vi "RT Main.vi"() -> ()   [LabVIEW 2016]
doc: "This template is for the Queued Message Handler design pattern.\n\nThe Event Handling Loop generates messages based on user interface actions.\n\nThe Message Handling Loop processes messages generated by the Event Handling Loop, or by other messages. The messages are string values, so new messages can be added easily to the Message Cases case structure in the Message Handling Loop. Each message cluster can also provide an optional value for Message Data, which is a variant that can be converted to whatever message-specific data is required."
uses:
  Globals/Global - All RT Loop Stop.vi
  Globals/Global - Monitoring Variables.vi
  Globals/Global - Configuration Options.vi
  Globals/Global - RT Stream Connections.vi
  <vilib>/FPGAPlugInAG/cRIO-9068/niLvFpga_Open_cRIO-9068.vi
  <vilib>/rvi/interface/common/dynamic/niFpgaDynamicAddResources.vi
  <vilib>/FPGAPlugInAG/Dynamic/niLvFpga_Reset_Dynamic.vi
  <vilib>/rvi/errors/niLvFpgaAdjustHostInterfaceError.vi
  <vilib>/FPGAPlugInAG/Dynamic/niLvFpga_Run_Dynamic.vi
  <vilib>/rvi/interface/nirviOpenFPGA/nirviOpenFPGA.xnode
  FPGA Bitfiles/v1.1.10032017CSU_FPGATarget2_FPGAMain_uXAbGLR-yyg.lvbitx
  FPGA Main.vi
  <vilib>/rvi/interface/nirviMethod/nirviMethod.xnode
  <vilib>/rvi/interface/nirviReadWriteControl/nirviReadWriteControl.xnode
  support/Message Queue/Message Queue.lvlib
  <vilib>/nisyscfg/nisyscfg.lvlib
  <vilib>/rvi/interface/Simulation/niFpgaSimulationCallBeginRW.vi
  NiFpgaLv.dll
panel:
  in  "error in (no error)":errorcluster
  # "Programa que contém a rotina principal do sistema.\nRoda todos os 4 loops principais;\nAquisição e armazenamento;\nSaúde do sistema e monitoramento da FPGA;\nComandos da interface de usuário;\nWatchdog.\n\nTambém contém a chamada para etapa de Transmissão, referente ao módulo NI 9269."
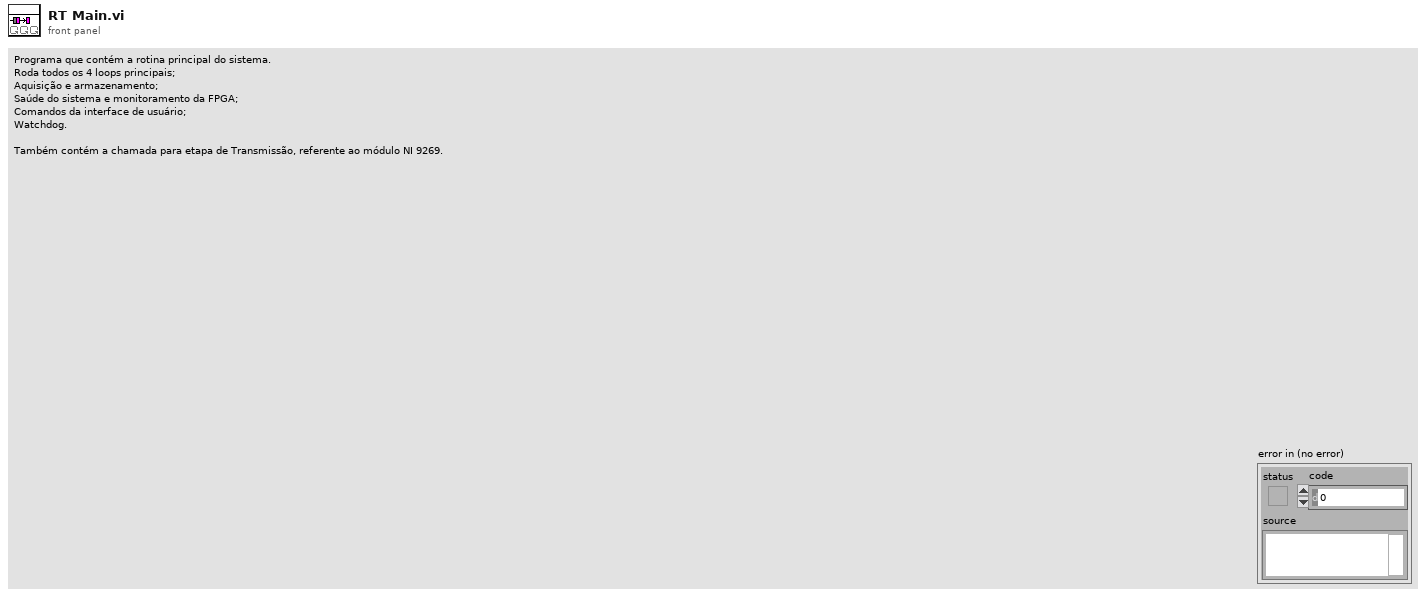
[diagram p1: front panel]
types:
  T1 = typedef "Acquisition and Logging Configuration.ctl" = cluster{"Data Rate":T2, "Samples per Read":i32, "Number of Reads to Save":i32, "Data File Name":string, "TDMS Properties":T3[], "Number of Channels":i32, "Channel Scale Array":fxp<+,24,12>[], "Channel Names":string[], "Trigger - RMS Value":dbl, "Trigger - Channel":i32, "Trigger - Time (Minute)":i32, "Frequency ":i32, "Amplitude (0~10)":dbl}
  T2 = typedef "nicrio_cRIO-9239_DataRatesRing.ctl" = u8
  T3 = typedef "TDMS Properties.ctl" = cluster{"Name":string, "Value":string}
  T4 = typedef "Message Queue.lvlib/All Real-Time Message Queues.ctl" = cluster{"Message Handler":refnum<queue>, "Acquisition and Logging":refnum<queue>}
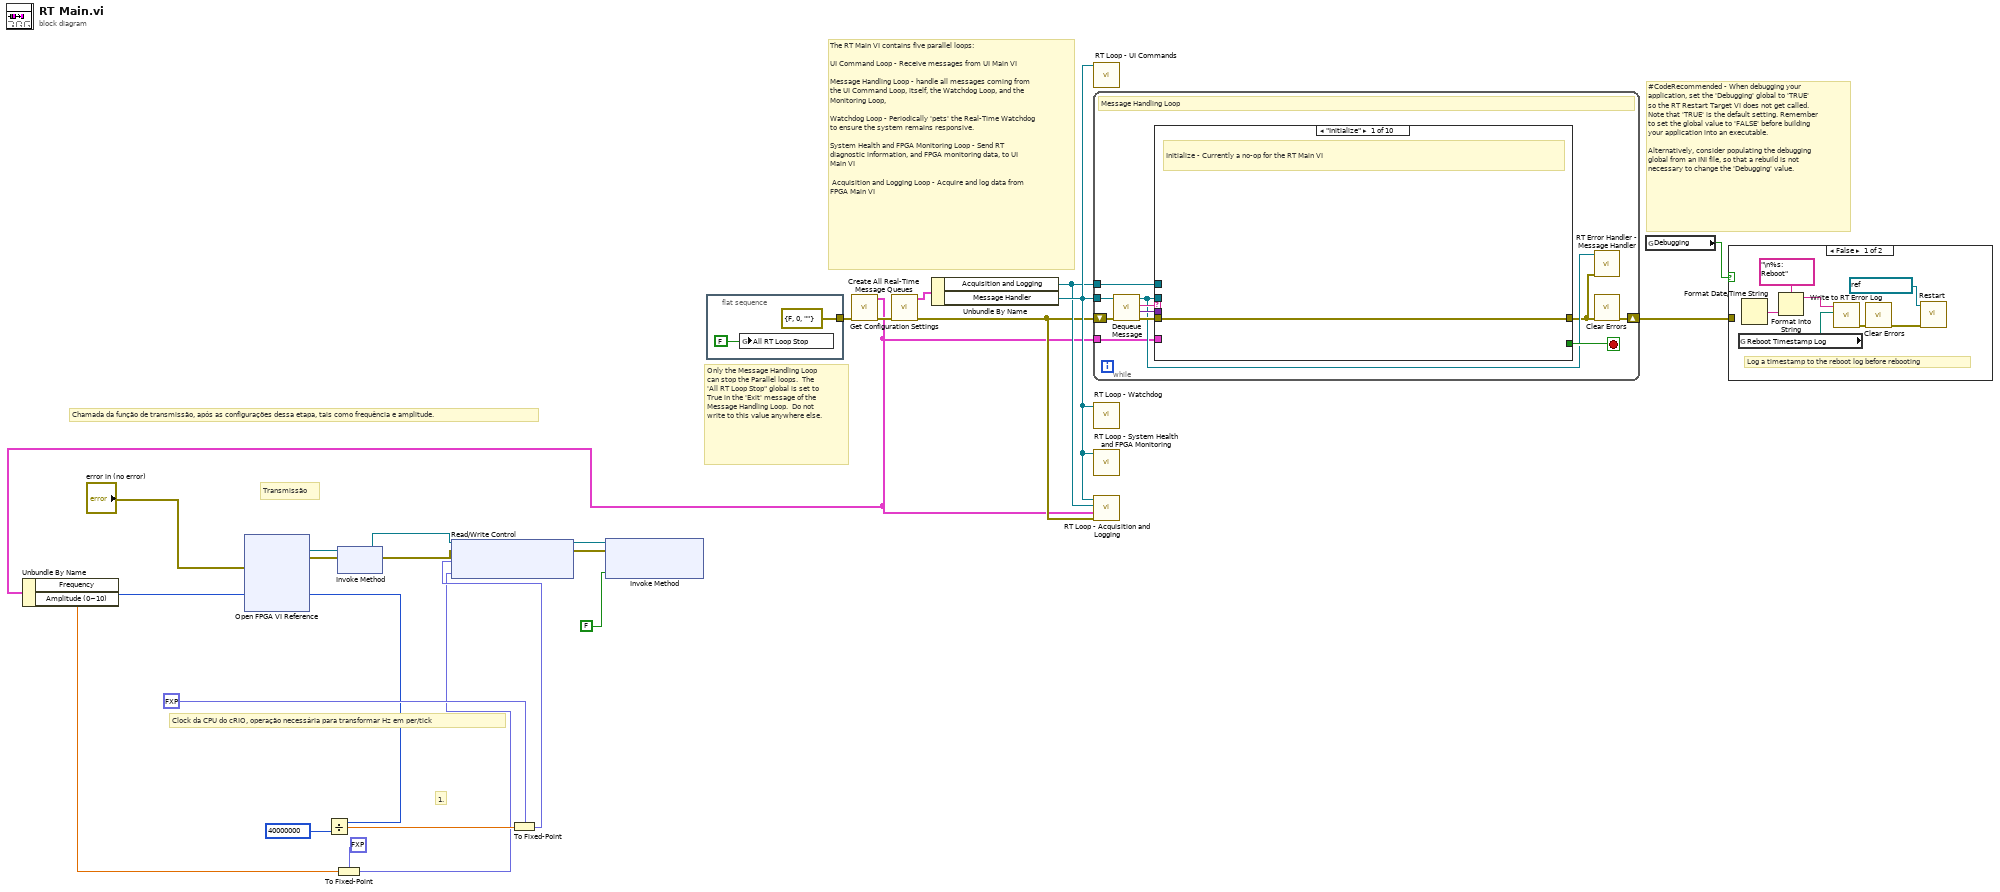
[diagram p0: block diagram]
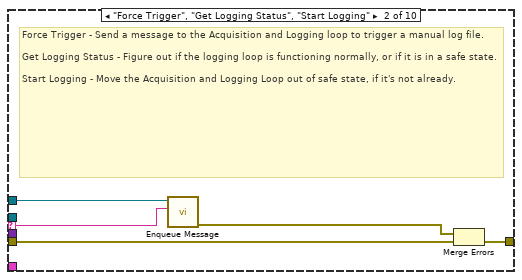
[diagram p3: hidden frame]
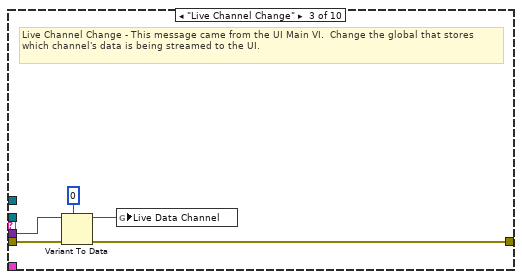
[diagram p4: hidden frame]
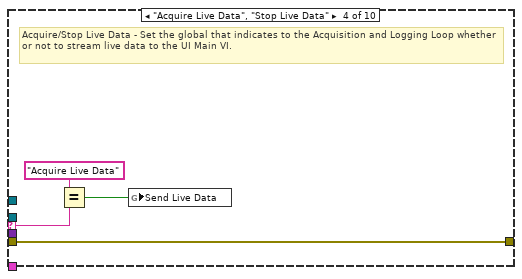
[diagram p5: hidden frame]
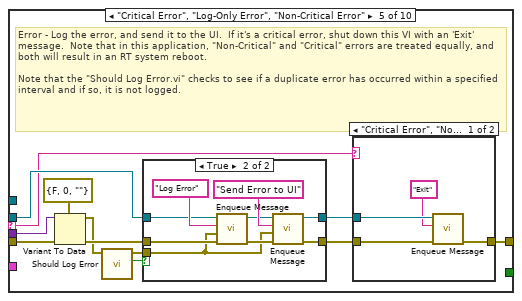
[diagram p6: hidden frame]
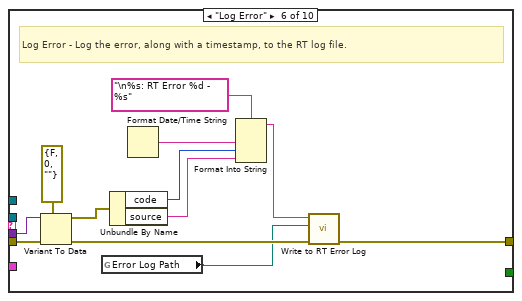
[diagram p9: hidden frame]
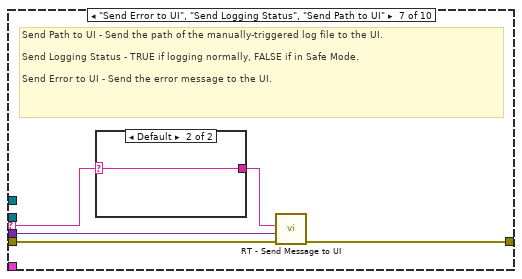
[diagram p10: hidden frame]
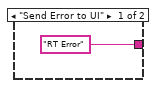
[diagram p11: hidden frame]
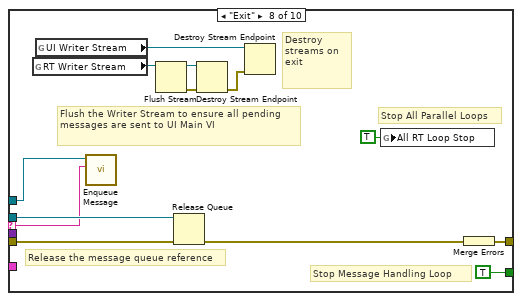
[diagram p12: hidden frame]
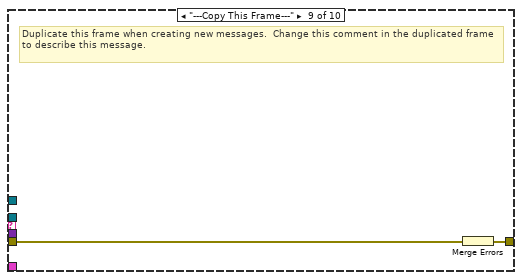
[diagram p13: hidden frame]
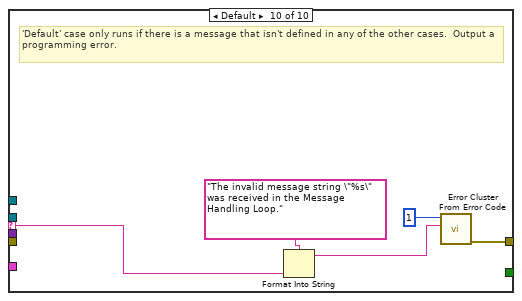
[diagram p14: hidden frame]
diagram:
  # "Chamada da função de transmissão, após as configurações dessa etapa, tais como frequência e amplitude."
  # "Transmissão"
  # "Clock da CPU do cRIO, operação necessária para transformar Hz em per/tick"
  # "1."
  # "#CodeRecommended - When debugging your application, set the 'Debugging' global to 'TRUE' so the RT Restart Target VI does not get called.  Note that 'TRUE' is the default setting. Remember to set the global value to 'FALSE' before building your application into an executable.\n\nAlternatively, consider populating the debugging global from an INI file, so that a rebuild is not necessary to change the 'Debugging' value."
  # "The RT Main VI contains five parallel loops:\n\nUI Command Loop - Receive messages from UI Main VI\n\nMessage Handling Loop - handle all messages coming from the UI Command Loop, itself, the Watchdog Loop, and the Monitoring Loop, \n\nWatchdog Loop - Periodically 'pets' the Real-Time Watchdog to ensure the system remains responsive.\n\nSystem Health and FPGA Monitoring Loop - Send RT diagnostic information, and FPGA monitoring data, to UI Main VI\n\n Acquisition and Logging Loop - Acquire and log data from FPGA Main VI"
  # "Only the Message Handling Loop can stop the Parallel loops.  The 'All RT Loop Stop\" global is set to True in the 'Exit' message of the Message Handling Loop.  Do not write to this value anywhere else."
  n1 = xnode "Open FPGA VI Reference"("error in"="error in (no error)") -> ("FPGA VI Reference Out"=w3:refnum<k20>, "error out"=w2:errorcluster)  [unwired: 1 in]
  n2 = xnode "Invoke Method"("FPGA VI Reference In"=w3, "error in"=w2) -> ("FPGA VI Reference Out"=w4:refnum<k20>, "error out"=w1:errorcluster)
  n3 = flat-sequence {
    tunnel: [errorcluster {"status"=FALSE, "code"=0, "source"=""} ("error constant")] -> w25
    frame #0 {
      n4 = global write "Global - All RT Loop Stop.vi" "All RT Loop Stop"(FALSE) -> ()
    }
  }
  n5 = call "Get Configuration Settings.vi"("error in (no error)"=w25) -> ("error out"=w22:errorcluster, "Acquisition and Logging Configuration"=w7:T1)  [unwired: 9 in]
  n6 = Unbundle By Name(w7) -> ("Frequency"=w5:i32, "Amplitude (0~10)"=w6:dbl)
  n7 = Divide(x=w5, y=40000000) -> (x/y=w15:dbl)
  n8 = To Fixed-Point(fixed-point type=fxp<+/-,20,5> 0.0, number=w6) -> (fixed-point=w12:fxp<+/-,20,5>)
  n9 = To Fixed-Point(fixed-point type=fxp<+,32,0> 0.0, number=w15) -> (fixed-point=w13:fxp<+,32,0>)
  n10 = xnode "Read/Write Control"("FPGA VI Reference In"=w4, "error in"=w1, "Frequency (periods/tick)"=w13, "Amplitude"=w12) -> ("FPGA VI Reference Out"=w11:refnum<k20>, "error out"=w10:errorcluster)
  n11 = xnode "Invoke Method"("FPGA VI Reference In"=w11, "error in"=w10, "Wait Until Done (F)"=FALSE) -> ()  [unwired: 2 out]
  n12 = call "Create All Real-Time Message Queues.vi"("error in (no error)"=w22) -> ("error out"=w18:errorcluster, "Message Queues out"=w20:T4)  [unwired: 9 in]
  n13 = Unbundle By Name(w20) -> ("Acquisition and Logging"=w19:refnum<queue>, "Message Handler"=w21:refnum<queue>)
  n14 = call "RT Loop - UI Commands.vi"("Message Queue"=w21) -> ()  [unwired: 11 in]
  n15 = while {
    tunnel: w21 -> [w33]
    shift-right: [w31] -> w24
    shift-left: w18 -> [w37]
    tunnel: w19 -> [w29]
    tunnel: w7 -> [w28]
    stop <- w38 stop-if-true
    # "Message Handling Loop"
    n16 = call "Dequeue Message.vi"("error in (no error)"=w37, "Message Queue"=w33) -> ("error out"=w36:errorcluster, "Message Data"=w34:variant, "Message"=w35:string, "dup Message Queue"=w32:refnum<queue>)  [unwired: 6 in]
    n17 = case "Message Cases" shown="\"Initialize\"" w35 {
      selector: w35 -> [_ w42 _ w52 w59 _ w95 w103 _ w119]
      tunnel: w32 -> [_ _ _ _ w60 _ _ w113 _ _]
      tunnel: w36 -> [w39 w44 w49 w53 w62 w93 w98 w109 w115 _]
      tunnel: [w39 w41 w48 w53 w65 w84 w97 w110 w114 w117] -> w30
      tunnel: [_ _ _ _ _ _ _ TRUE _ _] -> w38
      tunnel: w34 -> [_ _ w47 _ w54 w92 w96 _ _ _]
      tunnel: w29 -> [_ w43 _ _ _ _ _ w104 _ _]
      tunnel: w28 -> [_ _ _ _ _ _ _ _ _ _]
      frame "Initialize" {
        # "Initialize - Currently a no-op for the RT Main VI"
      }
      frame "Force Trigger", "Get Logging Status", "Start Logging" {
        # "Force Trigger - Send a message to the Acquisition and Logging loop to trigger a manual log file.\n\nGet Logging Status - Figure out if the logging loop is functioning normally, or if it is in a safe state.\n\nStart Logging - Move the Acquisition and Logging Loop out of safe state, if it's not already."
        n18 = call "Enqueue Message.vi"("Message"=w42, "Message Queue"=w43) -> ("error out"=w40:errorcluster)  [unwired: 8 in, 1 out]
        n19 = Merge Errors(w40, w44) -> (w41:errorcluster)
      }
      frame "Live Channel Change" {
        # "Live Channel Change - This message came from the UI Main VI.  Change the global that stores which channel's data is being streamed to the UI."
        n20 = Variant To Data(error in=w49, type=u32 0, Variant=w47) -> (data=w45:u32, error out=w48:errorcluster)
        n21 = global write "Global - Monitoring Variables.vi" "Live Data Channel"(w45) -> ()
      }
      frame "Acquire Live Data", "Stop Live Data" {
        # "Acquire/Stop Live Data - Set the global that indicates to the Acquisition and Logging Loop whether or not to stream live data to the UI Main VI."
        n22 = Equal?(x="Acquire Live Data", y=w52) -> (x = y?=w50:bool)
        n23 = global write "Global - Monitoring Variables.vi" "Send Live Data"(w50) -> ()
      }
      frame "Critical Error", "Log-Only Error", "Non-Critical Error" {
        # "Error - Log the error, and send it to the UI.  If it's a critical error, shut down this VI with an 'Exit' message.  Note that in this application, \"Non-Critical\" and \"Critical\" errors are treated equally, and both will result in an RT system reboot.\n\nNote that the \"Should Log Error.vi\" checks to see if a duplicate error has occurred within a specified interval and if so, it is not logged."
        n24 = Variant To Data(error in=w62, type=errorcluster {"status"=FALSE, "code"=0, "source"=""} ("error out"), Variant=w54) -> (data=w57:errorcluster, error out=w63:errorcluster)
        n25 = call "Should Log Error.vi"("error to report"=w57) -> ("Should Log Error?"=w55:bool, "dup error to report"=w56:errorcluster)  [unwired: 9 in]
        n26 = case shown="True" w55 {
          tunnel: [w67 w74] -> w61
          tunnel: [w66 w73] -> w58
          tunnel: w60 -> [w66 w72]
          tunnel: w63 -> [w67 w69]
          tunnel: w56 -> [_ w68]
          frame False {
          }
          frame True {
            n27 = call "Enqueue Message.vi"("error in (no error)"=w69, "Message Data"=w68, "Message"="Log Error", "Message Queue"=w72) -> ("error out"=w70:errorcluster, "dup Message Queue"=w71:refnum<queue>)  [unwired: 6 in]
            n28 = call "Enqueue Message.vi"("error in (no error)"=w70, "Message Data"=w68, "Message"="Send Error to UI", "Message Queue"=w71) -> ("error out"=w74:errorcluster, "dup Message Queue"=w73:refnum<queue>)  [unwired: 6 in]
          }
        }
        n29 = case shown="\"Critical Error\", \"Non-Critical Error\"" w59 {
          tunnel: w61 -> [w80 w81]
          tunnel: w58 -> [w78 _]
          tunnel: [w79 w81] -> w65
          frame "Critical Error", "Non-Critical Error" {
            n30 = call "Enqueue Message.vi"("error in (no error)"=w80, "Message"="Exit", "Message Queue"=w78) -> ("error out"=w79:errorcluster)  [unwired: 7 in, 1 out]
          }
          frame Default {
          }
        }
      }
      frame "Log Error" {
        # "Log Error - Log the error, along with a timestamp, to the RT log file."
        n31 = Variant To Data(error in=w93, type=errorcluster {"status"=FALSE, "code"=0, "source"=""} ("error constant"), Variant=w92) -> (data=w87:errorcluster, error out=w90:errorcluster)
        n32 = global read "Global - Configuration Options.vi" "Error Log Path"() -> (w82:path)
        n33 = Unbundle By Name(w87) -> ("code"=w86:i32, "source"=w85:string)
        n34 = Format Date/Time String() -> (date/time string=w88:string)  [unwired: 3 in]
        n35 = Format Into String(format string="\n%s: RT Error %d - %s", w88, w86, w85) -> (resulting string=w83:string)  [unwired: 2 in, 1 out]
        n36 = call "Write to RT Error Log.vi"("error in (no error)"=w90, "Error Log Path"=w82, "Log Entry"=w83) -> ("error out"=w84:errorcluster)  [unwired: 8 in]
      }
      frame "Send Error to UI", "Send Logging Status", "Send Path to UI" {
        # "Send Path to UI - Send the path of the manually-triggered log file to the UI.\n\nSend Logging Status - TRUE if logging normally, FALSE if in Safe Mode.\n\nSend Error to UI - Send the error message to the UI."
        n37 = case shown="Default" w95 {
          selector: w95 -> [_ w100]
          tunnel: ["RT Error" ("Message") w100] -> w94
          frame "Send Error to UI" {
          }
          frame Default {
          }
        }
        n38 = call "RT - Send Message to UI.vi"("error in (no error)"=w98, "Message Data"=w96, "Message"=w94) -> ("error out"=w97:errorcluster)  [unwired: 8 in]
      }
      frame "Exit" {
        # "Flush the Writer Stream to ensure all pending messages are sent to UI Main VI"
        # "Destroy streams on exit"
        # "Stop Message Handling Loop"
        # "Stop All Parallel Loops"
        # "Release the message queue reference"
        n39 = global read "Global - RT Stream Connections.vi" "RT Writer Stream"() -> (w107:refnum<k21>)
        n40 = global read "Global - RT Stream Connections.vi" "UI Writer Stream"() -> (w106:refnum<k21>)
        n41 = call "Enqueue Message.vi"("Message"=w103, "Message Queue"=w104) -> ()  [unwired: 8 in, 2 out]
        n42 = Flush Stream(11:w107) -> (0:w101:errorcluster, 3:w102:refnum<k21>)  [unwired: 3 in, 1 out]
        n43 = Release Queue(queue=w113, error in (no error)=w109) -> (error out=w111:errorcluster)  [unwired: 1 in, 2 out]
        n44 = Destroy Stream Endpoint(8:w101, 11:w102) -> (0:w105:errorcluster)
        n45 = Destroy Stream Endpoint(8:w105, 11:w106) -> ()  [unwired: 1 out]
        n46 = global write "Global - All RT Loop Stop.vi" "All RT Loop Stop"(TRUE ("Stop Monitoring Loops")) -> ()
        n47 = Merge Errors(w111) -> (w110:errorcluster)
      }
      frame "---Copy This Frame---" {
        # "Duplicate this frame when creating new messages.  Change this comment in the duplicated frame to describe this message."
        n48 = Merge Errors(w115) -> (w114:errorcluster)
      }
      frame Default {
        # "'Default' case only runs if there is a message that isn't defined in any of the other cases.  Output a programming error."
        n49 = Format Into String(format string="The invalid message string \"%s\" was received in the Message Handling Loop." ("Unknown Message Error Text"), w119) -> (resulting string=w116:string)  [unwired: 2 in, 1 out]
        n50 = call <vilib>:"Error Cluster From Error Code.vi"("error message (\"\")"=w116, "error code (0)"=1) -> ("error out"=w117:errorcluster)  [unwired: 7 in]
      }
    }
    n51 = call "RT Error Handler - Message Handler.vi"("error in (no error)"=w30, "Message Queue"=w32) -> ()  [unwired: 9 in, 1 out]
    n52 = call <vilib>:"Clear Errors.vi"("error in (no error)"=w30) -> ("error out"=w31:errorcluster)  [unwired: 5 in, 1 out]
  }
  n53 = call "RT Loop - Watchdog.vi"("Message Queue"=w21) -> ()  [unwired: 11 in]
  n54 = call "RT Loop - System Health and FPGA Monitoring.vi"("Message Queue"=w21) -> ()  [unwired: 11 in]
  n55 = call "RT Loop - Acquisition and Logging.vi"("error in (no error)"=w18, "Acquisition and Logging Configuration"=w7, "Acquisition and Logging Queue"=w19, "Message Queue"=w21) -> ()  [unwired: 8 in]
  n56 = global read "Global - Configuration Options.vi" "Debugging"() -> (w23:bool)
  n57 = case shown="False" w23 {
    tunnel: w24 -> [_ _]
    frame False {
      # "Log a timestamp to the reboot log before rebooting"
      n58 = global read "Global - Configuration Options.vi" "Reboot Timestamp Log"() -> (w123:path)
      n59 = Format Date/Time String() -> (date/time string=w125:string)  [unwired: 3 in]
      n60 = Format Into String(format string="\n%s: Reboot", w125) -> (resulting string=w124:string)  [unwired: 2 in, 1 out]
      n61 = call "Write to RT Error Log.vi"("Error Log Path"=w123, "Log Entry"=w124) -> ("error out"=w127:errorcluster)  [unwired: 9 in]
      n62 = call <vilib>:"Clear Errors.vi"("error in (no error)"=w127) -> ("error out"=w122:errorcluster)  [unwired: 5 in, 1 out]
      n63 = call <vilib>:"Restart.vi"("error in (no error)"=w122, "Session in"=refnum<k21> "localhost" ("session in")) -> ()  [unwired: 7 in, 3 out]
    }
    frame True {
    }
  }
